vi "RDV-getDataToMap.vi"(8 "error in (no error)":errorcluster, 11 "RDV-Reflection_Data_viewer in":refnum<class "RDV-Reflection_Data_viewer.lvclass">) -> (0 "error out":errorcluster, 1 "data":T2[](array[typedef]), 2 "all data":cluster{"key":string, "data":T1}[](array[cluster]), 3 "RDV-Reflection_Data_viewer out":refnum<class "RDV-Reflection_Data_viewer.lvclass">)   [LabVIEW 2020, in "RDV-Reflection_Data_viewer.lvclass"]
doc: "Returns the data clusters and the key/data pairs held in the viewer's data map."
uses:
  RDV-Reflection_Data_viewer.lvclass
  Reflector/RFH-common_data_format.ctl
  RDV-DATA_MAP_CLUST.ctl
  RDV-Reflection_Data_viewer.lvclass/RDV-Reflection_Data_viewer.ctl
  Reflector/RFH-Reflection_File_Handler.lvlib
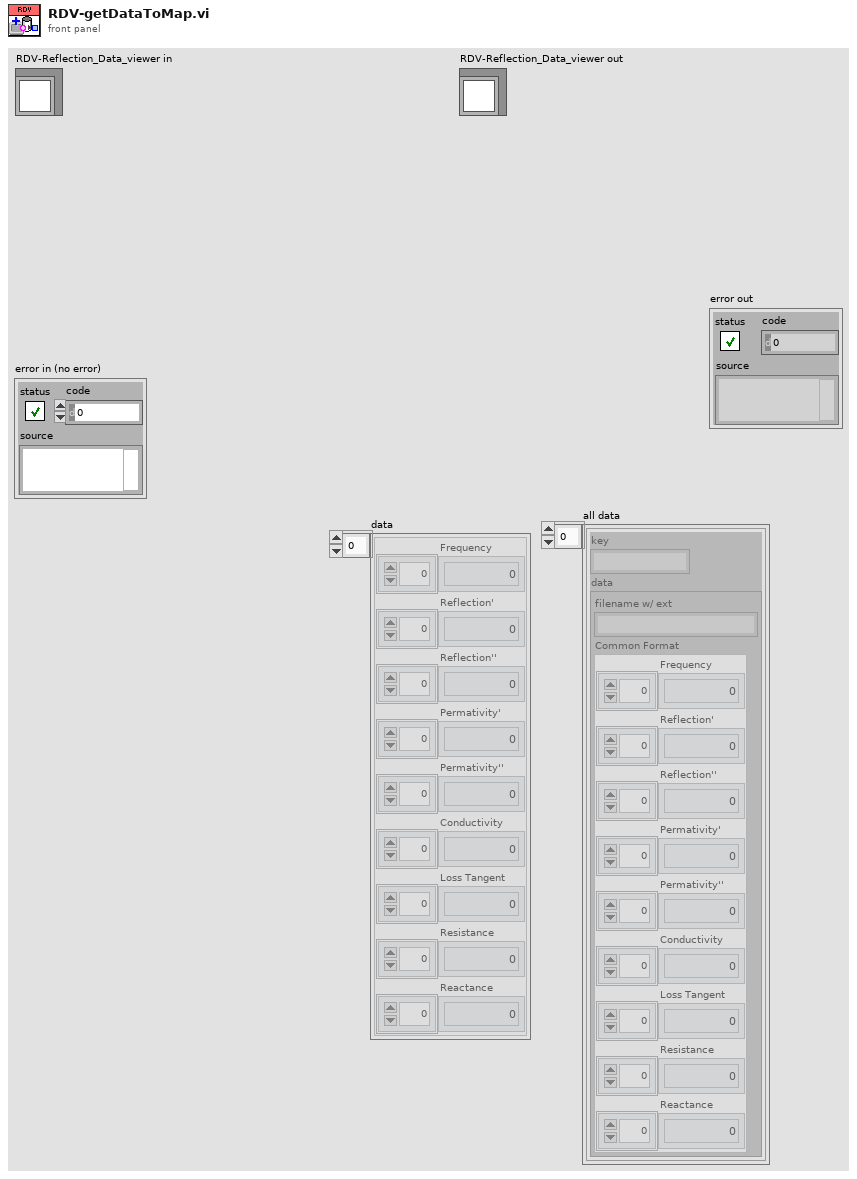
[diagram p1: front panel]
types:
  T1 = typedef "RDV-Reflection_Data_viewer.lvclass/RDV-DATA_MAP_CLUST.ctl" = cluster{"filename w/ ext":string, "Common Format":T2}
  T2 = typedef "RFH-Reflection_File_Handler.lvlib/RFH-common_data_format.ctl" = cluster{"Frequency":dbl[], "Reflection'":dbl[], "Reflection''":dbl[], "Permativity'":dbl[], "Permativity''":dbl[], "Conductivity":dbl[], "Loss Tangent":dbl[], "Resistance":dbl[], "Reactance":dbl[]}
  T3 = typedef "RDV-Reflection_Data_viewer.lvclass/RDV-DATA_MAP.ctl" = map{string, T1}
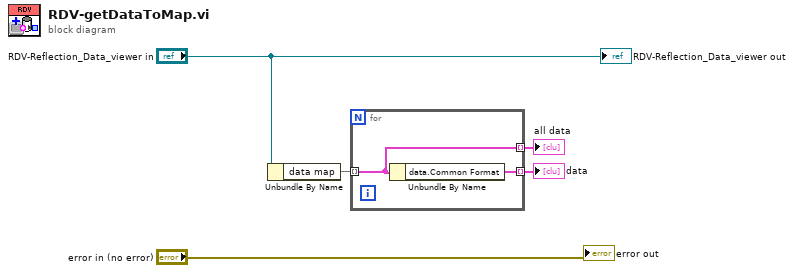
[diagram p0: block diagram]
diagram:
  n1 = Unbundle By Name("RDV-Reflection_Data_viewer in") -> ("data map"=w3:T3)
  n2 = for {
    tunnel: w3 -> [w6] mode=indexing
    tunnel: [w7] -> w2 mode=indexing
    tunnel: [w6] -> w1 mode=indexing
    n3 = Unbundle By Name(w6) -> ("data.Common Format"=w7:T2)
  }
  "data" <- w2
  "all data" <- w1
  "error out" <- "error in (no error)"
  "RDV-Reflection_Data_viewer out" <- "RDV-Reflection_Data_viewer in"
